vi "Measurement Logic.vi"(8 "error in":errorcluster, 9 "measurement configuration":T2={"CAPTURING STREAM"=FALSE, "INTERFACE NAME STRING"="", "ETHERNET MODE IN"=0, "INTERFACE NAME"="ENET9/monitor"}, 10 "measure call context in":refnum<class "Measure Call Context.lvclass">, 11 "Stop OOB Server UE":refnum<user-event>) -> (0 "error out":errorcluster, 1 "measurement results":T1, 2 "measure call context out":refnum<class "Measure Call Context.lvclass">)   [LabVIEW 2025, in "Automotive Ethernet Bus Monitor.lvclass"]
doc: "Contains the core logic for executing the measurement."
uses:
  Automotive Ethernet Bus Monitor.lvclass
  <vilib>/Plug-In SDKs/Measurements/Measure Call Context/Measure Call Context.lvclass
  Measurement Configuration.ctl
  Measurement Results.ctl
  Logic Data.ctl
  State.ctl
  Buffer/Create Frame Buffer.vi
  <vilib>/xnet/xnet.llb/XNET Create Session (Frame Input Stream).vi
  <vilib>/xnet/xnet.llb/XNET Read (Frame Ethernet).vi
  Buffer/Enqueue Frame.vi
  Buffer/Destroy Frame Buffer.vi
  Automotive Ethernet Bus Monitor.lvclass/Automotive Ethernet Bus Monitor.ctl
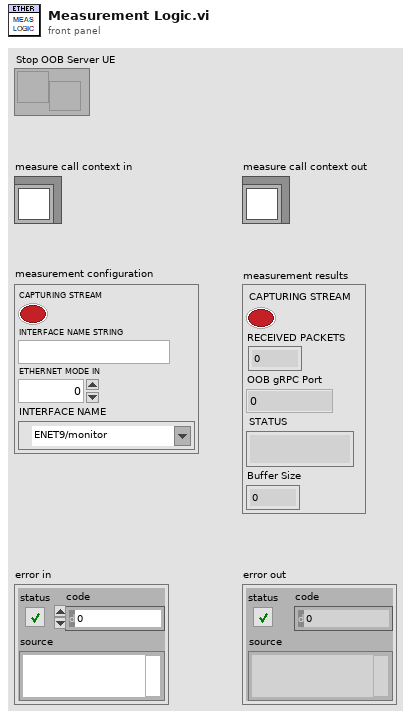
[diagram p1: front panel]
types:
  T1 = typedef "Automotive Ethernet Bus Monitor.lvclass/Measurement Results.ctl" = cluster{"CAPTURING STREAM":bool, "RECEIVED PACKETS":i32, "OOB gRPC Port":i32, "STATUS":string, "Buffer Size":i32}
  T2 = typedef "Automotive Ethernet Bus Monitor.lvclass/Measurement Configuration.ctl" = cluster{"CAPTURING STREAM":bool, "INTERFACE NAME STRING":string, "ETHERNET MODE IN":i32, "INTERFACE NAME":refnum<k21>}
  T3 = typedef "Automotive Ethernet Bus Monitor.lvclass/Logic Data.ctl" = cluster{"State":T4, "Results":T1, "Session":refnum<k21>, "Rows":i32, "Frames":string[][]}
  T4 = typedef "Automotive Ethernet Bus Monitor.lvclass/State.ctl" = enum16{"Init", "Execute", "Results", "Error", "Close"}
  T5 = typedef "XNET Frame Ethernet.ctl" = cluster{"local timestamp":timestamp, "network timestamp":timestamp, "frame data":u8[], "fcs":u32, "type":T6, "network synced?":bool, "receive?":bool, "transmit?":bool, "error?":bool}
  T6 = typedef "XNET Frame Type Ethernet.ctl" = u16
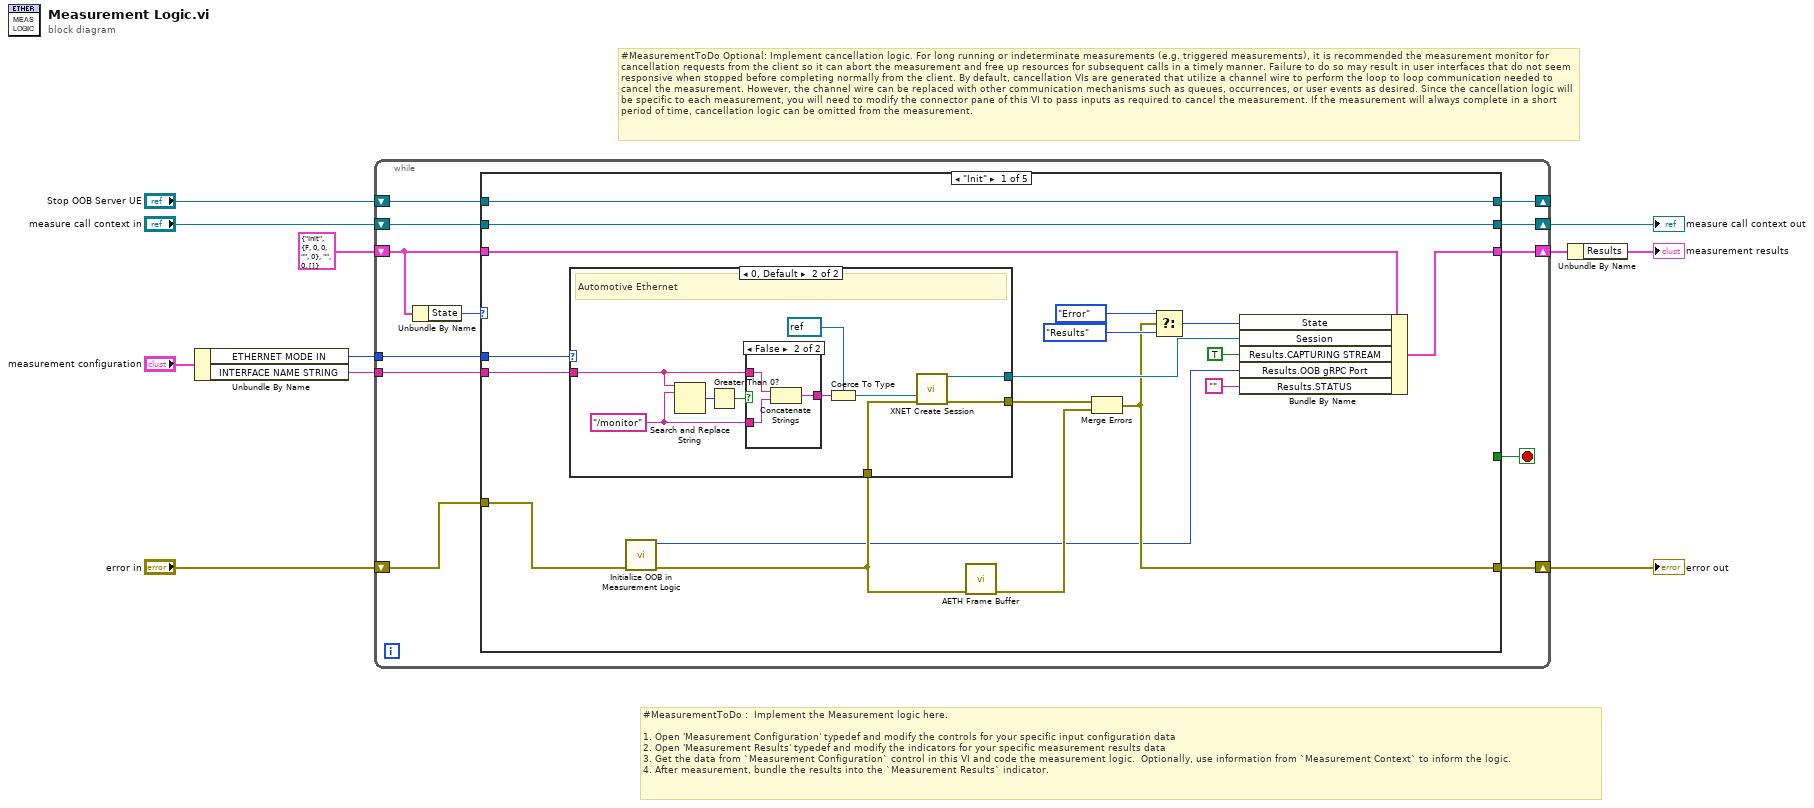
[diagram p0: block diagram]
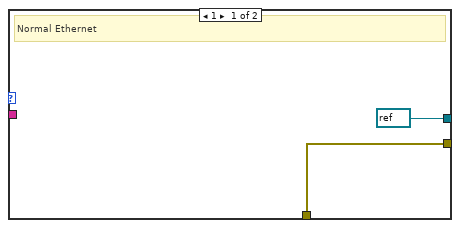
[diagram p2: hidden frame]
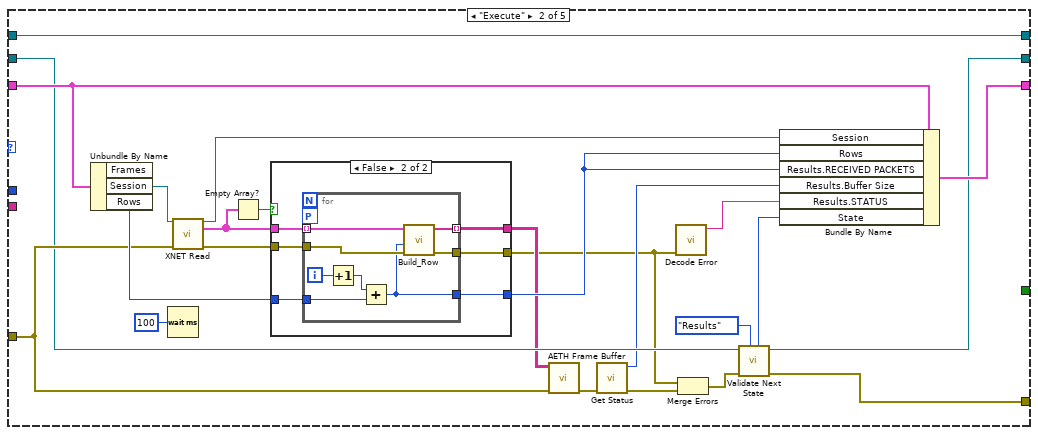
[diagram p4: hidden frame]
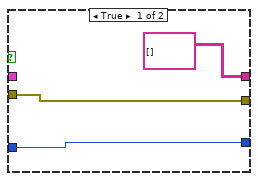
[diagram p5: hidden frame]
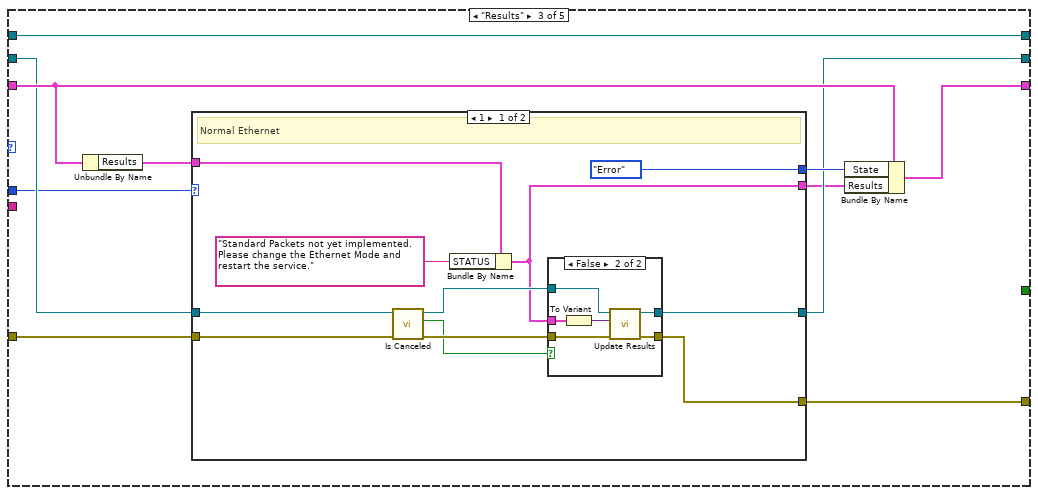
[diagram p6: hidden frame]
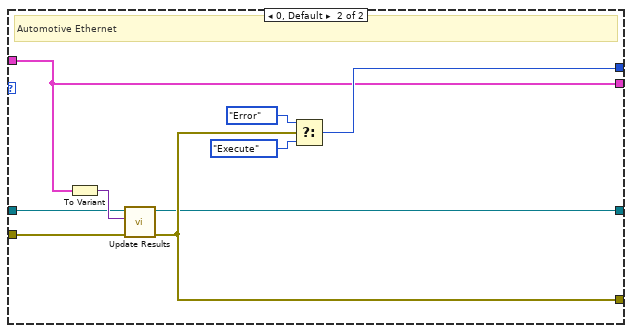
[diagram p8: hidden frame]
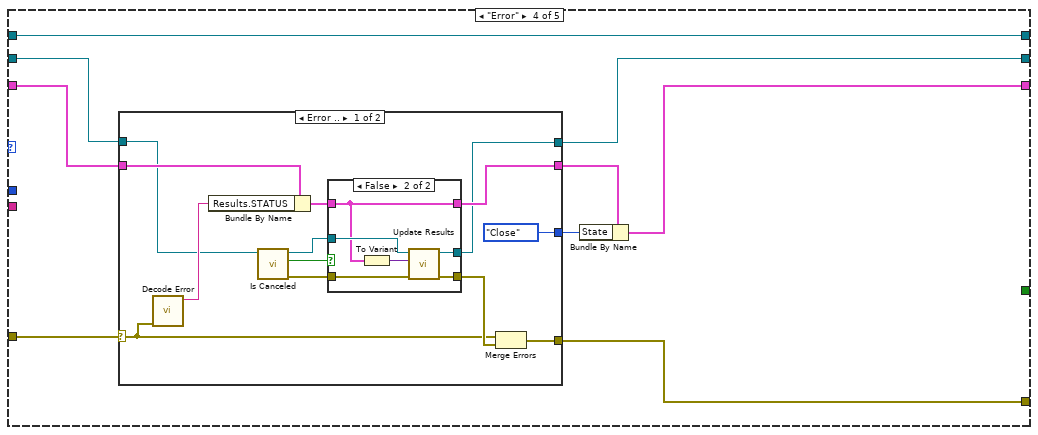
[diagram p9: hidden frame]
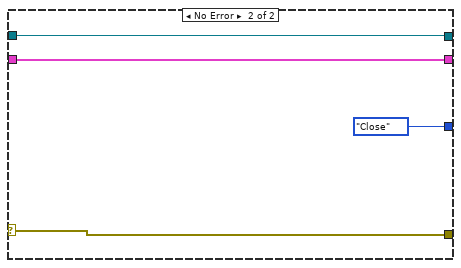
[diagram p11: hidden frame]
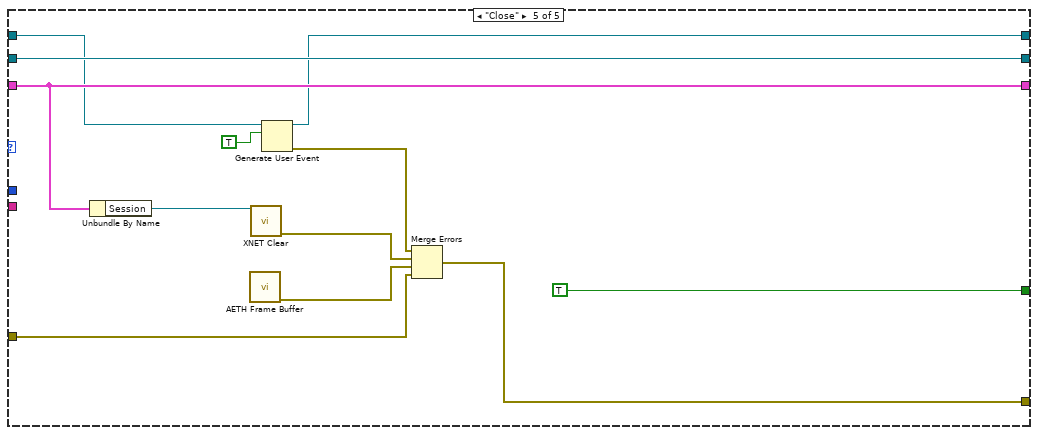
[diagram p12: hidden frame]
diagram:
  # "#MeasurementToDo Optional: Implement cancellation logic. For long running or indeterminate measurements (e.g. triggered measurements), it is recommended the measurement monitor for cancellation requests from the client so it can abort the measurement and free up resources for subsequent calls in a timely manner. Failure to do so may result in user interfaces that do not seem responsive when stopped before completing normally from the client. By default, cancellation VIs are generated that utilize a channel wire to perform the loop to loop communication needed to cancel the measurement. However, the channel wire can be replaced with other communication mechanisms such as queues, occurrences, or user events as desired. Since the cancellation logic will be specific to each measurement, you will need to modify the connector pane of this VI to pass inputs as required to cancel the measurement. If the measurement will always complete in a short period of time, cancellation logic can be omitted from the measurement."
  # "#MeasurementToDo :  Implement the Measurement logic here.\n\n1. Open 'Measurement Configuration' typedef and modify the controls for your specific input configuration data\n2. Open 'Measurement Results' typedef and modify the indicators for your specific measurement results data\n3. Get the data from `Measurement Configuration` control in this VI and code the measurement logic.  Optionally, use information from `Measurement Context` to inform the logic.\n4. After measurement, bundle the results into the `Measurement Results` indicator."
  n1 = Unbundle By Name("measurement configuration") -> ("ETHERNET MODE IN"=w2:i32, "INTERFACE NAME STRING"=w10:string)
  n2 = while {
    tunnel: w10 -> [w21]
    shift-right: [w20] -> w5
    shift-left: "error in" -> [w19]
    shift-right: [w18] -> w4
    shift-left: T3 {"State"=enum."Init", "Results"={"CAPTURING STREAM"=FALSE, "RECEIVED PACKETS"=0, "OOB gRPC Port"=0, "STATUS"="", "Buffer Size"=0}, "Session"="", "Rows"=0, "Frames"=[]} ("Logic Data") -> [w23]
    shift-right: [w17] -> w6
    shift-left: "measure call context in" -> [w16]
    shift-right: [w13] -> _
    shift-left: "Stop OOB Server UE" -> [w14]
    tunnel: w2 -> [w12]
    stop <- w15 stop-if-true
    n3 = Unbundle By Name(w23) -> ("State"=w22:T4)
    n4 = case shown="\"Init\"" w22 {
      tunnel: w23 -> [w40 w74 w107 w144 w182]
      tunnel: w21 -> [w41 _ _ _ _]
      tunnel: [w27 w70 w105 w146 w180] -> w20
      tunnel: w19 -> [w32 w72 w104 w145 w174]
      tunnel: [w39 w79 w109 w143 w182] -> w18
      tunnel: [w34 w68 w103 w141 w183] -> w17
      tunnel: w16 -> [w34 w69 w102 w139 w183]
      tunnel: [_ _ _ _ TRUE] -> w15
      tunnel: w14 -> [w31 w73 w101 w138 w179]
      tunnel: [w31 w73 w101 w138 w178] -> w13
      tunnel: w12 -> [w25 _ w100 _ _]
      frame "Init" {
        n5 = call "Initialize OOB in Measurement Logic.vi"("error in"=w32) -> ("error out"=w30:errorcluster, "OBB Port"=w26:i32)  [unwired: 9 in]
        n6 = case shown="0, Default" w25 {
          tunnel: w41 -> [_ w50]
          tunnel: [refnum<k21> refnum ("session out") w46] -> w38
          tunnel: w30 -> [w42 w45]
          tunnel: [w42 w44] -> w28
          frame 1 {
            # "Normal Ethernet"
          }
          frame 0, Default {
            w51 = "/monitor" ("string")
            # "Automotive Ethernet"
            n7 = Search and Replace String(input string=w50, search string=w51) -> (number of replacements=w52:i32)  [unwired: 6 in, 3 out]
            n8 = Greater Than 0?(x=w52) -> (x > 0?=w53:bool)
            n9 = case shown="False" w53 {
              tunnel: w50 -> [w54 w57]
              tunnel: w51 -> [_ w56]
              tunnel: [w54 w55] -> w48
              frame True {
              }
              frame False {
                n10 = Concatenate Strings(w57, w56) -> (w55:string)
              }
            }
            n11 = Coerce To Type(0:w48, 1:refnum<k21> refnum ("interface")) -> (2:w47:refnum<k21>)
            n12 = call-poly <vilib>:"XNET Create Session.vi"("interface"=w47, "error in (no error)"=w45) -> ("session out"=w46:refnum<k21>, "error out"=w44:errorcluster)  [unwired: 12 in]
          }
        }
        n13 = call-poly "AETH Frame Buffer.vi"("error in"=w30) -> ("error out"=w29:errorcluster)  [unwired: 10 in]
        n14 = Merge Errors(w28, w29) -> (w27:errorcluster)
        n15 = Select(t=State."Error" ("State"), s=w27, f=State."Results" ("State")) -> (s? t:f=w35:T4)
        n16 = Bundle By Name(cluster=w40, "State"=w35, "Session"=w38, "Results.CAPTURING STREAM"=TRUE, "Results.OOB gRPC Port"=w26, "Results.STATUS"="") -> (w39:T3)
      }
      frame "Execute" {
        n17 = Unbundle By Name(w74) -> ("Session"=w80:refnum<k21>, "Rows"=w75:i32)  [unwired: 1 out]
        n18 = Wait (ms)(milliseconds to wait=u32 100) -> ()  [unwired: 1 out]
        n19 = call-poly <vilib>:"XNET Read.vi"("session in"=w80, "error in (no error)"=w72) -> ("session out"=w58:refnum<k21>, "data"=w78:T5[], "error out"=w76:errorcluster)  [unwired: 10 in, 1 out]
        n20 = Empty Array?(array=w78) -> (empty?=w77:bool)
        n21 = case shown="False" w77 {
          tunnel: w78 -> [_ w90]
          tunnel: w76 -> [w83 w89]
          tunnel: w75 -> [w84 w88]
          tunnel: [w84 w87] -> w67
          tunnel: [w83 w86] -> w61
          tunnel: [string[][] [] ("Packet") w85] -> w63
          frame True {
          }
          frame False {
            n22 = for {
              tunnel: w90 -> [w97] mode=indexing
              tunnel: w88 -> [w92]
              tunnel: [w93] -> w87
              tunnel: w89 -> [w96]
              tunnel: [w95] -> w86
              tunnel: [w94] -> w85 mode=indexing
              workers-P: _ -> [_]
              i -> [w98]
              n23 = Increment(x=w98) -> (x+1=w91:i32)
              n24 = Add(x=w91, y=w92) -> (x+y=w93:i32)
              n25 = call "Build_Row.vi"("error in (no error)"=w96, "Packet Number"=w93, "Ethernet frame"=w97) -> ("error out"=w95:errorcluster, "Packet"=w94:string[])  [unwired: 7 in]
            }
          }
        }
        n26 = call-poly "AETH Frame Buffer.vi"("error in"=w72, "Data"=w63) -> ("error out"=w71:errorcluster)  [unwired: 8 in, 1 out]
        n27 = call "Get Status.vi"("error in"=w71) -> ("error out"=w65:errorcluster, "Messages"=w66:i32)  [unwired: 9 in]
        n28 = call "Decode Error.vi"("Error In"=w61) -> ("Status Message"=w59:string)  [unwired: 10 in]
        n29 = Merge Errors(w61, w65) -> (w64:errorcluster)
        n30 = call "Validate Next State.vi"("Normal State"=State."Results" ("State"), "error in"=w64, "Measure Call Context in"=w69) -> ("error out"=w70:errorcluster, "measure call context out"=w68:refnum<class "Measure Call Context.lvclass">, "Next State"=w60:T4)  [unwired: 6 in]
        n31 = Bundle By Name(cluster=w74, "Session"=w58, "Rows"=w67, "Results.RECEIVED PACKETS"=w67, "Results.Buffer Size"=w66, "Results.STATUS"=w59, "State"=w60) -> (w79:T3)
      }
      frame "Results" {
        n32 = Unbundle By Name(w107) -> ("Results"=w106:T1)
        n33 = case shown="1" w100 {
          tunnel: [State."Error" ("State") w135] -> w108
          tunnel: w106 -> [w111 w129]
          tunnel: [w116 w133] -> w105
          tunnel: w104 -> [w114 w132]
          tunnel: [w115 w131] -> w103
          tunnel: w102 -> [w112 w130]
          tunnel: [w110 w129] -> w99
          frame 1 {
            # "Normal Ethernet"
            n34 = call <vilib>:"Is Canceled.vi"("error in"=w114, "measure call context in"=w112) -> ("error out"=w119:errorcluster, "is canceled?"=w118:bool, "measure call context out"=w120:refnum<class "Measure Call Context.lvclass">)  [unwired: 7 in]
            n35 = Bundle By Name(cluster=w111, "STATUS"="Standard Packets not yet implemented. Please change the Ethernet Mode and restart the service.") -> (w110:T1)
            n36 = case shown="False" w118 {
              tunnel: w120 -> [w122 w125]
              tunnel: w119 -> [w121 w124]
              tunnel: w110 -> [_ w127]
              tunnel: [w122 w126] -> w115
              tunnel: [w121 w123] -> w116
              frame True {
              }
              frame False {
                n37 = To Variant(anything=w127) -> (Variant=w128:variant)
                n38 = call <vilib>:"Update Results.vi"("error in"=w124, "measurement results"=w128, "measure call context in"=w125) -> ("error out"=w123:errorcluster, "measure call context out"=w126:refnum<class "Measure Call Context.lvclass">)  [unwired: 7 in]
              }
            }
          }
          frame 0, Default {
            # "Automotive Ethernet"
            n39 = To Variant(anything=w129) -> (Variant=w134:variant)
            n40 = call <vilib>:"Update Results.vi"("error in"=w132, "measurement results"=w134, "measure call context in"=w130) -> ("error out"=w133:errorcluster, "measure call context out"=w131:refnum<class "Measure Call Context.lvclass">)  [unwired: 7 in]
            n41 = Select(t=State."Error", s=w133, f=State."Execute" ("State")) -> (s? t:f=w135:T4)
          }
        }
        n42 = Bundle By Name(cluster=w107, "State"=w108, "Results"=w99) -> (w109:T3)
      }
      frame "Error" {
        n43 = case shown="Error .." w145 {
          selector: w145 -> [w151 w171]
          tunnel: w144 -> [w156 w170]
          tunnel: [w152 w171] -> w146
          tunnel: [w150 w170] -> w140
          tunnel: [State."Close" ("State") State."Close" ("State")] -> w142
          tunnel: [w148 w169] -> w141
          tunnel: w139 -> [w147 w169]
          frame Error {
            n44 = call "Decode Error.vi"("Error In"=w151) -> ("Status Message"=w155:string)  [unwired: 10 in]
            n45 = Bundle By Name(cluster=w156, "Results.STATUS"=w155) -> (w154:T3)
            n46 = call <vilib>:"Is Canceled.vi"("measure call context in"=w147) -> ("error out"=w157:errorcluster, "is canceled?"=w159:bool, "measure call context out"=w158:refnum<class "Measure Call Context.lvclass">)  [unwired: 8 in]
            n47 = case shown="False" w159 {
              tunnel: w154 -> [w160 w163]
              tunnel: [w161 w168] -> w153
              tunnel: w157 -> [w161 w167]
              tunnel: w158 -> [w162 w166]
              tunnel: [w162 w165] -> w148
              tunnel: [w160 w163] -> w150
              frame True {
              }
              frame False {
                n48 = To Variant(anything=w163) -> (Variant=w164:variant)
                n49 = call <vilib>:"Update Results.vi"("error in"=w167, "measurement results"=w164, "measure call context in"=w166) -> ("error out"=w168:errorcluster, "measure call context out"=w165:refnum<class "Measure Call Context.lvclass">)  [unwired: 7 in]
              }
            }
            n50 = Merge Errors(w151, w153) -> (w152:errorcluster)
          }
          frame No Error {
          }
        }
        n51 = Bundle By Name(cluster=w140, "State"=w142) -> (w143:T3)
      }
      frame "Close" {
        n52 = Unbundle By Name(w182) -> ("Session"=w173:refnum<k21>)
        n53 = call-poly "AETH Frame Buffer.vi"() -> ("error out"=w175:errorcluster)  [unwired: 11 in]
        n54 = call <vilib>:"XNET Clear.vi"("session in"=w173) -> ("error out"=w176:errorcluster)  [unwired: 14 in]
        n55 = Generate User Event(user event=w179, event data cluster=TRUE ("event data")) -> (user event out=w178:refnum<user-event>, error out=w177:errorcluster)  [unwired: 2 in]
        n56 = Merge Errors(w177, w176, w175, w174) -> (w180:errorcluster)
      }
    }
  }
  "error out" <- w5
  "measure call context out" <- w6
  n57 = Unbundle By Name(w4) -> ("Results"=→"measurement results":T1)
